vi "set Modulation.vi"(8 "error in (no error)":errorcluster, 10 "Modulation":T1, 11 "NR in":refnum<class "NR.lvclass">) -> (0 "error out":errorcluster, 3 "NR out":refnum<class "NR.lvclass">)   [LabVIEW 2023, in "ANRITSU Call Box.lvlib" / "NR.lvclass"]
uses:
  NR.lvclass
  Type Definition/NR Modulation Type.ctl
  ANRITSU Call Box.lvlib
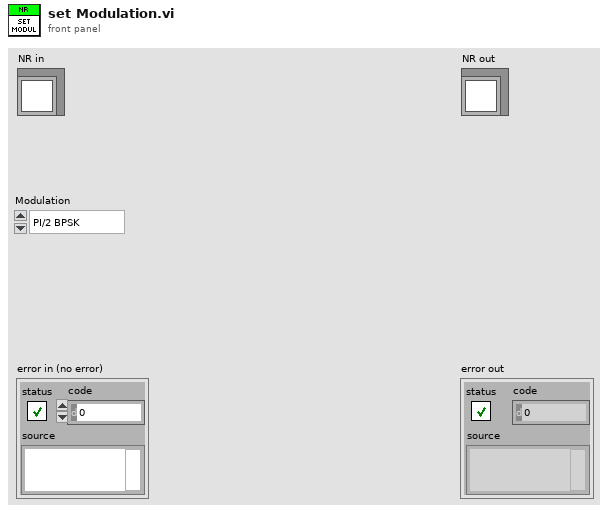
[diagram p1: front panel]
types:
  T1 = typedef "ANRITSU Call Box.lvlib/NR Modulation Type.ctl" = enum16{"PI/2 BPSK", "QPSK", "16QAM", "64QAM", "256QAM"}
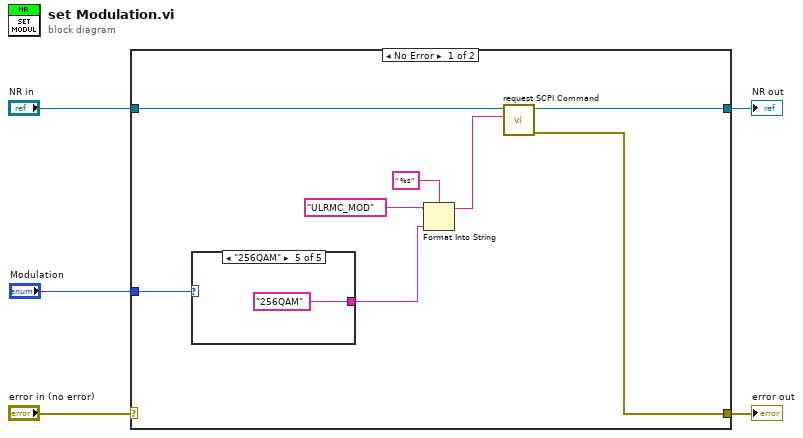
[diagram p0: block diagram]
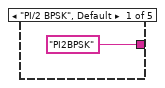
[diagram p2: hidden frame]
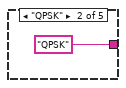
[diagram p3: hidden frame]
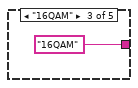
[diagram p4: hidden frame]
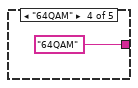
[diagram p5: hidden frame]
diagram:
  n1 = case shown="No Error" "error in (no error)" {
    selector: "error in (no error)" -> [_ w20]
    tunnel: [w6 w20] -> w4
    tunnel: [w7 w19] -> w2
    tunnel: "NR in" -> [w9 w19]
    tunnel: "Modulation" -> [w10 _]
    frame No Error {
      n2 = case shown="\"256QAM\"" w10 {
        tunnel: ["PI2BPSK" ("initial string") "QPSK" ("initial string") "16QAM" ("initial string") "64QAM" ("initial string") "256QAM" ("initial string")] -> w11
        frame "PI/2 BPSK", Default {
        }
        frame "QPSK" {
        }
        frame "16QAM" {
        }
        frame "64QAM" {
        }
        frame "256QAM" {
        }
      }
      n3 = Format Into String(format string=" %s", initial string="ULRMC_MOD", w11) -> (resulting string=w8:string)  [unwired: 1 in, 1 out]
      n4 = call "request SCPI Command.vi"("SCPI Command"=w8, "NR in"=w9) -> ("error out"=w6:errorcluster, "NR out"=w7:refnum<class "NR.lvclass">)  [unwired: 8 in]
    }
    frame Error {
    }
  }
  "error out" <- w4
  "NR out" <- w2
